vi "RemoteVI Announce Listener.vi"(0 "stop notifier name":string, 5 "listener result":errorcluster) -> ()   [LabVIEW 2020, in "RemoteVI.lvlib"]
doc: "Tells RemoteVI Start.vi whether the server is listening: sends listener result (the error cluster of TCP Create Listener) on the notifier named <stop notifier name>:started and releases it. Start.vi has obtained that notifier before it launched the loop and waits on it, so a port in use is reported to the caller."
uses:
  RemoteVI.lvlib
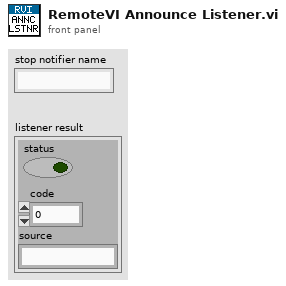
[diagram p1: front panel]
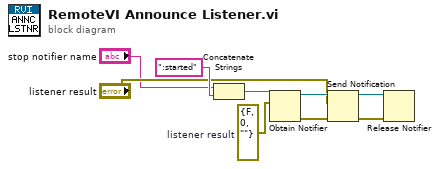
[diagram p0: block diagram]
diagram:
  w5 = errorcluster {"status"=FALSE, "code"=0, "source"=""}  # listener result
  n1 = Concatenate Strings("stop notifier name", ":started") -> (w4:string)
  n2 = Obtain Notifier(name (unnamed)=w4, notification data type=w5) -> (notifier out=w6:refnum<notifier>, error out=w7:errorcluster)  [unwired: 2 in, 1 out]
  n3 = Send Notification(notification="listener result", notifier=w6, error in (no error)=w7) -> (notifier out=w8:refnum<notifier>, error out=w9:errorcluster)
  n4 = Release Notifier(notifier=w8, error in (no error)=w9) -> ()  [unwired: 1 in, 3 out]
